vi "Test MQTT-3.1.2-3.vi"(8 "error in (no error)":errorcluster, 11 "Connection Config":refnum<class "Connection.lvclass">) -> (0 "error out":errorcluster, 3 "Connection Config dup":refnum<class "Connection.lvclass">)   [LabVIEW 2013]
uses:
  <vilib>/LabVIEW Open Source Project/MQTT Control Packets/Control Packets/CONNECT/CONNECT.lvclass
  <vilib>/LabVIEW Open Source Project/MQTT Control Packets/Control Packets/ControlPacket/ControlPacket.lvclass
  <vilib>/addons/_JKI Toolkits/Caraya/classes/Test/Test.lvclass
  <vilib>/LabVIEW Open Source Project/Connection/Connection/Connection.lvclass
  <vilib>/addons/_JKI Toolkits/Caraya/classes/Assert/Assert.lvclass
  <vilib>/addons/_JKI Toolkits/Caraya/classes/Assert/Assert Equal Value_Variant.vi
  <vilib>/LabVIEW Open Source Project/MQTT Connection/MQTT_Connection/Connection/Connection.lvclass
panel:
  out "timed out":bool
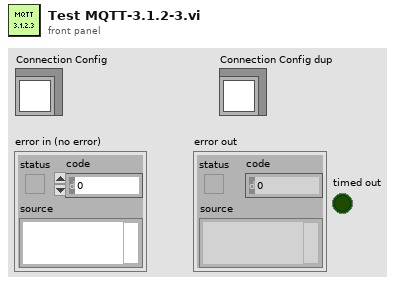
[diagram p1: front panel]
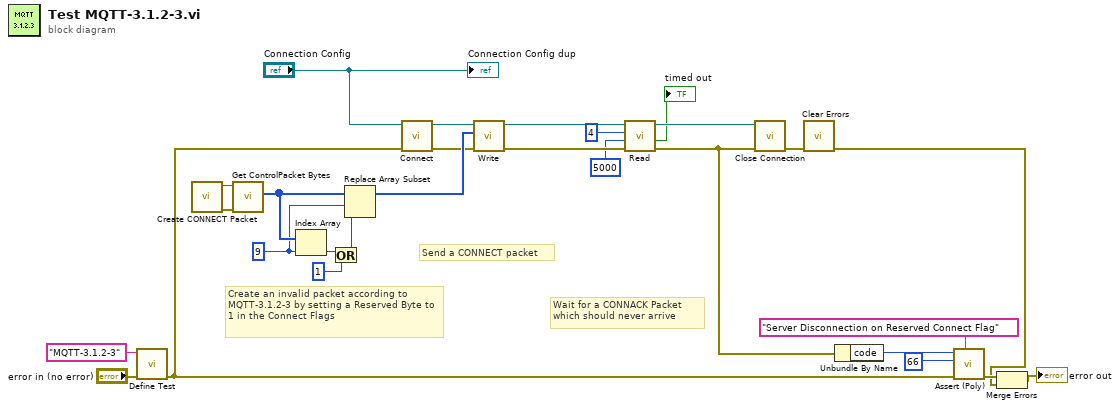
[diagram p0: block diagram]
diagram:
  w20 = 9 ("index")
  # "Wait for a CONNACK Packet\nwhich should never arrive"
  # "Create an invalid packet according to MQTT-3.1.2-3 by setting a Reserved Byte to 1 in the Connect Flags"
  # "Send a CONNECT packet"
  n1 = call <vilib>:"Define Test.vi"("error in (no error)"="error in (no error)", "Label (VI Title)"="MQTT-3.1.2-3") -> ("error out"=w4:errorcluster)  [unwired: 9 in]
  n2 = call <vilib>:"Create CONNECT Packet.vi"() -> ("error out"=w27:errorcluster, "CONNECT"=w28:refnum<class "CONNECT.lvclass">)  [unwired: 9 in, 1 out]
  n3 = call <vilib>:"Get ControlPacket Bytes.vi"("error in (no error)"=w27, "ControlPacket"=w28) -> ("Bytes Stream"=w22:u8[])  [unwired: 6 in, 3 out]
  n4 = Index Array(array=w22, index=w20) -> (element=w24:u8)
  n5 = Or(x=w24, y=u8 1) -> (x .or. y?=w19:u8)
  n6 = Replace Array Subset(array=w22, new element=w19, index=w20) -> (w21:u8[])
  n7 = call <vilib>:"Connect.vi"("error in (no error)"=w4, "Connection in"="Connection Config") -> ("error out"=w5:errorcluster, "Connection out"=w6:refnum<class "Connection.lvclass">)  [unwired: 8 in]
  n8 = call <vilib>:"Write.vi"("error in (no error)"=w5, "Bytes"=w21, "Connection in"=w6) -> ("error out"=w25:errorcluster, "Connection"=w26:refnum<class "Connection.lvclass">)  [unwired: 7 in]
  n9 = call <vilib>:"Read.vi"("error in (no error)"=w25, "timeout (2000 ms)"=5000 ("timeout ms (25000)"), "bytes to read (100)"=4 ("bytes to read"), "TCPConnection in"=w26) -> ("error out"=w8:errorcluster, "timed out"=→"timed out":bool, "TCPConnection out"=w18:refnum<class "Connection.lvclass">)  [unwired: 3 in, 2 out]
  n10 = call <vilib>:"Close Connection.vi"("error in (no error)"=w8, "Connection in"=w18) -> ("error out"=w12:errorcluster)  [unwired: 8 in, 1 out]
  n11 = call <vilib>:"Clear Errors.vi"("error in (no error)"=w12) -> ("error out"=w7:errorcluster)  [unwired: 6 in]
  n12 = Unbundle By Name(w8) -> ("code"=w3:i32)
  n13 = call-poly <vilib>:"Assert (Poly).vi"("Label"="Server Disconnection on Reserved Connect Flag", "error in (no error)"=w4, "Y"=66 ("code"), "X"=w3) -> ("error out"=w16:errorcluster)  [unwired: 7 in]
  n14 = Merge Errors(w16, w7) -> (→"error out":errorcluster)
  "Connection Config dup" <- "Connection Config"
